vi "Test_Render.vi"() -> ()   [LabVIEW 2026]
doc: "UI_Render 테스트: 화면을 PNG로 저장."
panel:
  out "error out":errorcluster
  in  "PNG Path":path
  in  "Status Text":string
  in  "Status":T1(ring)=enum."Player Turn"
  in  "Stones":i32[](array[numeric])=[1, 2]
  in  "Cols":i32[](array[numeric])=[7, 8]
  in  "Rows":i32[](array[numeric])=[7, 7]
  in  "Hover Button":i32=-1
  in  "Settings":i32[](array[numeric])=[0, 0, 1, 1]
  in  "Screen":enum16{"Settings", "Game"}(ring)
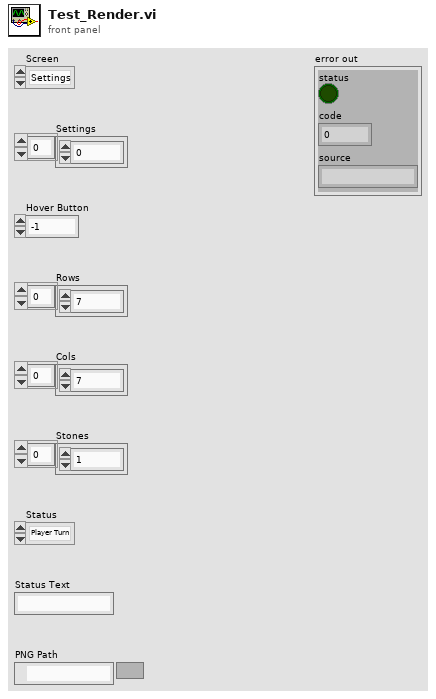
[diagram p1: front panel]
types:
  T1 = enum16{"Idle", "Player Turn", "AI Thinking", "Game Over"}
  T2 = cluster{"left":i16, "top":i16, "right":i16, "bottom":i16}
  T3 = cluster{"Screen":enum16{"Settings", "Game"}, "Settings":i32[], "Board":cluster{"Grid":enum8{"Empty", "Black", "White"}[][], "Move History":cluster{"Row":i32, "Col":i32, "Stone":enum8{"Empty", "Black", "White"}}[], "Last Move":cluster{"Row":i32, "Col":i32, "Stone":enum8{"Empty", "Black", "White"}}}, "Status":enum16{"Idle", "Player Turn", "AI Thinking", "Game Over"}, "Game ID":u32, "Player Stone":enum8{"Empty", "Black", "White"}, "Hover":cluster{"Row":i32, "Col":i32, "Stone":enum8{"Empty", "Black", "White"}}, "Hover Button":i32, "Win Line":cluster{"Row":i32, "Col":i32, "Stone":enum8{"Empty", "Black", "White"}}[], "Score 1":i32, "Score 2":i32, "Draws":i32, "Status Text":string, "Status Color":u32}
  T4 = cluster{"Grid":enum8{"Empty", "Black", "White"}[][], "Move History":cluster{"Row":i32, "Col":i32, "Stone":enum8{"Empty", "Black", "White"}}[], "Last Move":cluster{"Row":i32, "Col":i32, "Stone":enum8{"Empty", "Black", "White"}}}
  T5 = cluster{"Row":i32, "Col":i32, "Stone":enum8{"Empty", "Black", "White"}}
  T6 = typedef "imagedata.ctl" = cluster{"image type":i32, "image depth":i32, "image":u8[], "mask":u8[], "colors":u32[], "Rectangle":cluster{"left":i16, "top":i16, "right":i16, "bottom":i16}}
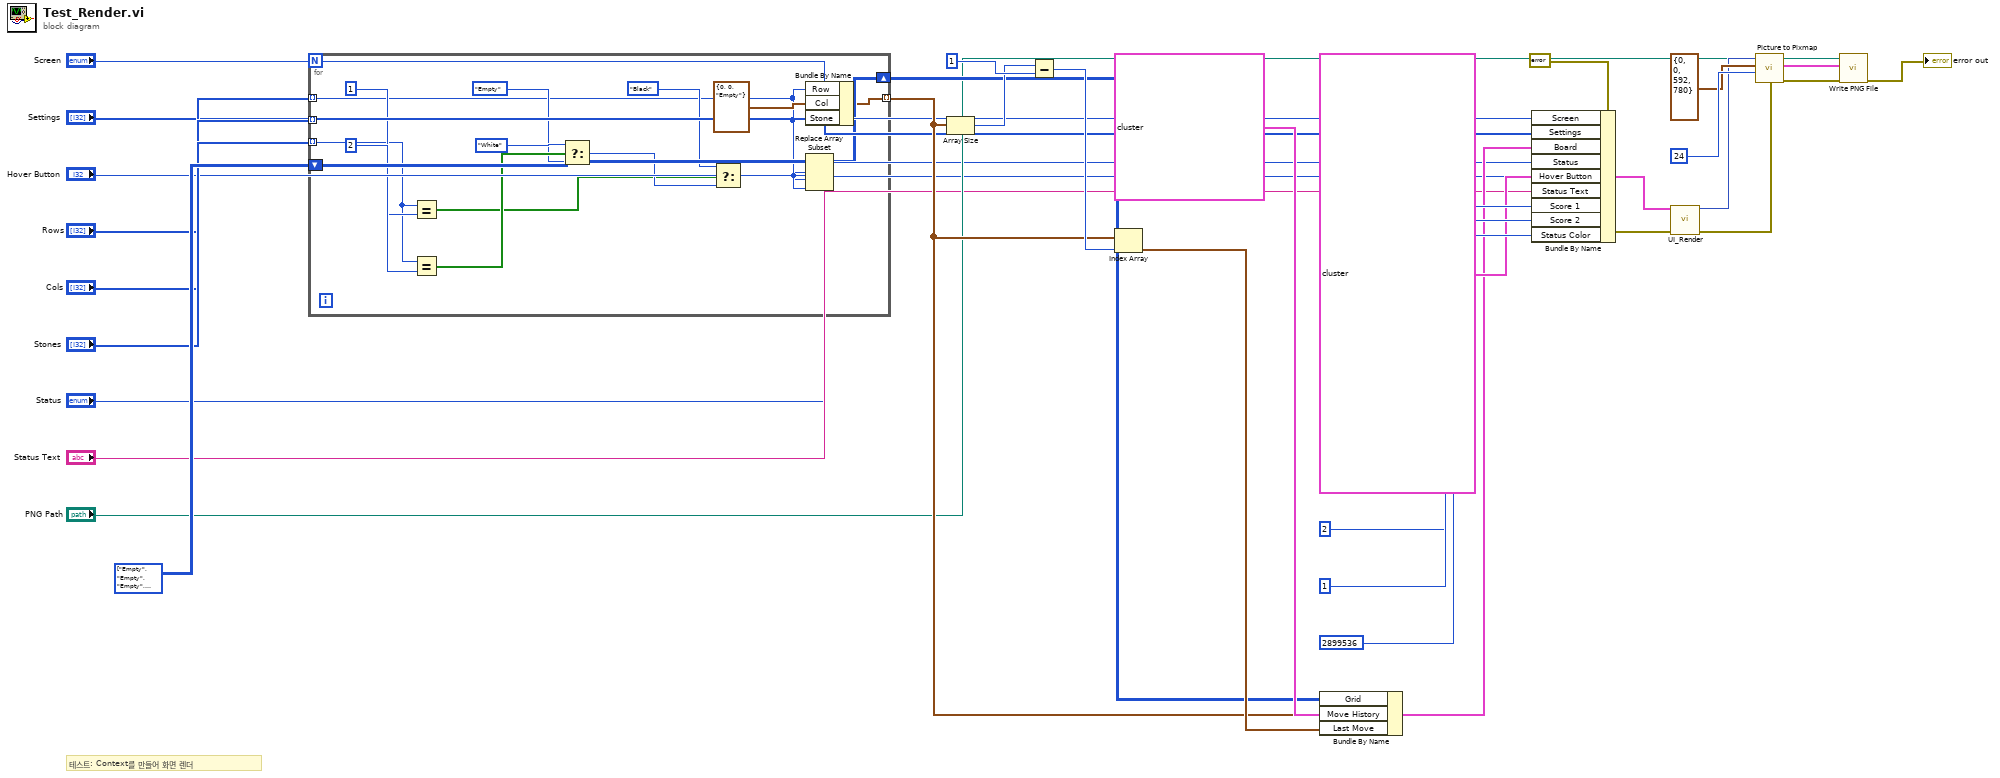
[diagram p0: block diagram]
diagram:
  w10 = enum8{"Empty", "Black", "White"}[][] [[enum."Empty", enum."Empty", enum."Empty", enum."Empty", enum."Empty", enum."Empty", enum."Empty", enum."Empty", enum."Empty", enum."Empty", enum."Empty", enum."Empty", enum."Empty", enum."Empty", enum."Empty"], [enum."Empty", enum."Empty", enum."Empty", enum."Empty", enum."Empty", enum."Empty", enum."Empty", enum."Empty", enum."Empty", enum."Empty", enum."Empty", enum."Empty", enum."Empty", enum."Empty", enum."Empty"], [enum."Empty", enum."Empty", enum."Empty", enum."Empty", enum."Empty", enum."Empty", enum."Empty", enum."Empty", enum."Empty", enum."Empty", enum."Empty", enum."Empty", enum."Empty", enum."Empty", enum."Empty"], [enum."Empty", enum."Empty", enum."Empty", enum."Empty", enum."Empty", enum."Empty", enum."Empty", enum."Empty", enum."Empty", enum."Empty", enum."Empty", enum."Empty", enum."Empty", enum."Empty", enum."Empty"], [enum."Empty", enum."Empty", enum."Empty", enum."Empty", enum."Empty", enum."Empty", enum."Empty", enum."Empty", enum."Empty", enum."Empty", enum."Empty", enum."Empty", enum."Empty", enum."Empty", enum."Empty"], [enum."Empty", enum."Empty", enum."Empty", enum."Empty", enum."Empty", enum."Empty", enum."Empty", enum."Empty", enum."Empty", enum."Empty", enum."Empty", enum."Empty", enum."Empty", enum."Empty", enum."Empty"], [enum."Empty", enum."Empty", enum."Empty", enum."Empty", enum."Empty", enum."Empty", enum."Empty", enum."Empty", enum."Empty", enum."Empty", enum."Empty", enum."Empty", enum."Empty", enum."Empty", enum."Empty"], [enum."Empty", enum."Empty", enum."Empty", enum."Empty", enum."Empty", enum."Empty", enum."Empty", enum."Empty", enum."Empty", enum."Empty", enum."Empty", enum."Empty", enum."Empty", enum."Empty", enum."Empty"], [enum."Empty", enum."Empty", enum."Empty", enum."Empty", enum."Empty", enum."Empty", enum."Empty", enum."Empty", enum."Empty", enum."Empty", enum."Empty", enum."Empty", enum."Empty", enum."Empty", enum."Empty"], [enum."Empty", enum."Empty", enum."Empty", enum."Empty", enum."Empty", enum."Empty", enum."Empty", enum."Empty", enum."Empty", enum."Empty", enum."Empty", enum."Empty", enum."Empty", enum."Empty", enum."Empty"], [enum."Empty", enum."Empty", enum."Empty", enum."Empty", enum."Empty", enum."Empty", enum."Empty", enum."Empty", enum."Empty", enum."Empty", enum."Empty", enum."Empty", enum."Empty", enum."Empty", enum."Empty"], [enum."Empty", enum."Empty", enum."Empty", enum."Empty", enum."Empty", enum."Empty", enum."Empty", enum."Empty", enum."Empty", enum."Empty", enum."Empty", enum."Empty", enum."Empty", enum."Empty", enum."Empty"], [enum."Empty", enum."Empty", enum."Empty", enum."Empty", enum."Empty", enum."Empty", enum."Empty", enum."Empty", enum."Empty", enum."Empty", enum."Empty", enum."Empty", enum."Empty", enum."Empty", enum."Empty"], [enum."Empty", enum."Empty", enum."Empty", enum."Empty", enum."Empty", enum."Empty", enum."Empty", enum."Empty", enum."Empty", enum."Empty", enum."Empty", enum."Empty", enum."Empty", enum."Empty", enum."Empty"], [enum."Empty", enum."Empty", enum."Empty", enum."Empty", enum."Empty", enum."Empty", enum."Empty", enum."Empty", enum."Empty", enum."Empty", enum."Empty", enum."Empty", enum."Empty", enum."Empty", enum."Empty"]] items=["Empty", "Black", "White"]
  # "테스트: Context를 만들어 화면 렌더"
  n1 = for {
    tunnel: "Rows" -> [w31] mode=indexing
    tunnel: "Cols" -> [w32] mode=indexing
    tunnel: "Stones" -> [w33] mode=indexing
    shift-right: [w45] -> w12
    shift-left: w10 -> [w46]
    tunnel: [w44] -> w11 mode=indexing
    n2 = Equal?(x=w33, y=1) -> (x = y?=w38:bool[])
    n3 = Equal?(x=w33, y=2) -> (x = y?=w40:bool[])
    n4 = Select(t=enum8{"Empty", "Black", "White"}."White", s=w40, f=enum8{"Empty", "Black", "White"}."Empty") -> (s? t:f=w41:enum8{"Empty", "Black", "White"})
    n5 = Select(t=enum8{"Empty", "Black", "White"}."Black", s=w38, f=w41) -> (s? t:f=w42:enum8{"Empty", "Black", "White"})
    n6 = Bundle By Name(cluster=T5 {"Row"=0, "Col"=0, "Stone"=enum."Empty"}, "Row"=w31, "Col"=w32, "Stone"=w42) -> (w44:T5)
    n7 = Replace Array Subset(array=w46, new element=w42, index (row)=w31, index (col)=w32) -> (w45:enum8{"Empty", "Black", "White"}[][])
  }
  n8 = Array Size(array=w11) -> (size(s)=w13:i32)
  n9 = Subtract(x=w13, y=1) -> (x-y=w15:i32)
  n10 = Index Array(array=w11, index=w15) -> (element=w16:T5)
  n11 = Bundle By Name(cluster=T4 {"Grid"=array15x15[225 elements], "Move History"=[], "Last Move"={"Row"=-1, "Col"=-1, "Stone"=enum."Empty"}}, "Grid"=w12, "Move History"=w11, "Last Move"=w16) -> (w18:T4)
  n12 = Bundle By Name(cluster=T3 {"Screen"=enum."Settings", "Settings"=[0, 0, 1, 1], "Board"={"Grid"=array15x15[225 elements], "Move History"=[], "Last Move"={"Row"=-1, "Col"=-1, "Stone"=enum."Empty"}}, "Status"=enum."Idle", "Game ID"=0, "Player Stone"=enum."Black", "Hover"={"Row"=-1, "Col"=-1, "Stone"=enum."Empty"}, "Hover Button"=-1, "Win Line"=[], "Score 1"=0, "Score 2"=0, "Draws"=0, "Status Text"="", "Status Color"=0}, "Screen"="Screen", "Settings"="Settings", "Board"=w18, "Status"="Status", "Hover Button"="Hover Button", "Status Text"="Status Text", "Score 1"=2, "Score 2"=1, "Status Color"=u32 2899536) -> (w23:T3)
  n13 = call "UI_Render.vi"("Context"=w23, "error in"=errorcluster {"status"=FALSE, "code"=0, "source"=""}) -> ("Picture"=w25:picture, "error out"=w26:errorcluster)  [unwired: 12 in]
  n14 = call <vilib>:"Picture to Pixmap.vi"("depth"=24, "rect"=T2 {"left"=0, "top"=0, "right"=592, "bottom"=780}, "picture"=w25) -> ("image data"=w29:T6)  [unwired: 7 in, 1 out]
  n15 = call <vilib>:"Write PNG File.vi"("error in (no error)"=w26, "image data"=w29, "path to PNG file"="PNG Path") -> ("error out"=→"error out":errorcluster)  [unwired: 7 in, 1 out]
